vi "Is Read Notify Enabled.vi"(8 "error in (no error)":errorcluster) -> (0 "error out":errorcluster, 2 "return type":u8)   [LabVIEW 2017, in "HID_ARZ.lvlib"]
doc: "IS_READ_NOTIFY_ENABLED IsReadNotifyEnabled;"
uses:
  HID_ARZ.lvlib
  <userlib>/HID_ARZ/mcHID.dll
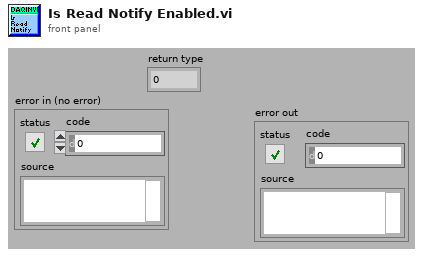
[diagram p1: front panel]
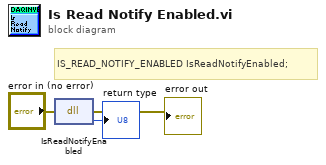
[diagram p0: block diagram]
diagram:
  # "IS_READ_NOTIFY_ENABLED IsReadNotifyEnabled;"
  n1 = dll-call lib="C:/Program Files (x86)/National Instruments/LabVIEW 2017/user.lib/HID_ARZ/mcHID.*" fn="IsReadNotifyEnabled"(error in="error in (no error)") -> (error out=→"error out":errorcluster, "return type"=→"return type":u8)  [unwired: 2 in, 1 out]
